vi "Read Commands.vi"(8 "error in (no error)":errorcluster, 11 "Iteration Actions in":refnum<class "Iteration Actions.lvclass">) -> (0 "error out":errorcluster, 1 "Analog Commands":map{refnum<class "MessageQ.lvclass">, T3}(c390), 2 "Digital Commands":map{refnum<class "MessageQ.lvclass">, T5}(c390), 3 "Iteration Actions out":refnum<class "Iteration Actions.lvclass">, 4 "Remote Analog":map{string, T1}(c390), 6 "Remote Digital":map{string, T2}(c390))   [LabVIEW 2020, in "VolatusSeq.lvlib" / "Iteration Actions.lvclass"]
uses:
  Iteration Actions.lvclass
  Volatus/MessageQ/MessageQ.lvclass
  messages/CmdDigitalMultiple/Data.ctl
  messages/CmdDigital/Data.ctl
  messages/CmdAnalogMultiple/Data.ctl
  messages/CmdAnalog/Data.ctl
  Iteration Actions.lvclass/Iteration Actions.ctl
  messages/CmdDigital/CmdDigital.lvlib
  messages/CmdDigitalMultiple/CmdDigitalMultiple.lvlib
  messages/CmdAnalog/CmdAnalog.lvlib
  messages/CmdAnalogMultiple/CmdAnalogMultiple.lvlib
  messages/CmdDigitalMultiple/Class/Msg.lvclass
  Remote Digital.ctl
  VolatusSeq.lvlib
  messages/CmdAnalogMultiple/Class/Msg.lvclass
  Remote Analog.ctl
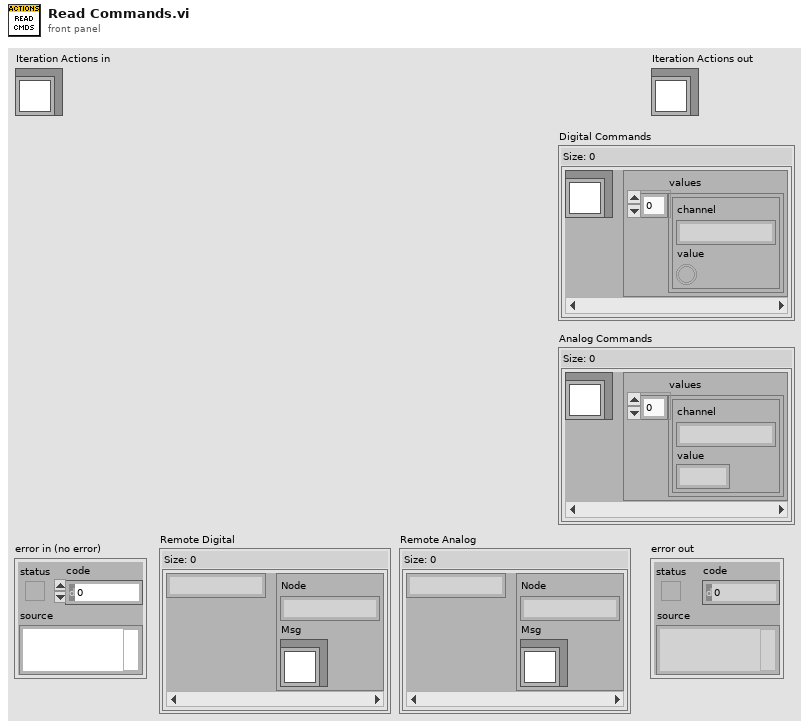
[diagram p1: front panel]
types:
  T1 = typedef "VolatusSeq.lvlib/Remote Analog.ctl" = cluster{"Node":string, "Msg":refnum<class "Msg.lvclass">}
  T2 = typedef "VolatusSeq.lvlib/Remote Digital.ctl" = cluster{"Node":string, "Msg":refnum<class "Msg.lvclass">}
  T3 = typedef "CmdAnalogMultiple.lvlib/Data.ctl" = cluster{"values":T4[]}
  T4 = typedef "CmdAnalog.lvlib/Data.ctl" = cluster{"channel":string, "value":dbl}
  T5 = typedef "CmdDigitalMultiple.lvlib/Data.ctl" = cluster{"values":T6[]}
  T6 = typedef "CmdDigital.lvlib/Data.ctl" = cluster{"channel":string, "value":bool}
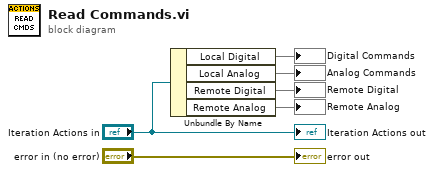
[diagram p0: block diagram]
diagram:
  n1 = Unbundle By Name("Iteration Actions in") -> ("Local Digital"=→"Digital Commands":map{refnum<class "MessageQ.lvclass">, T5}, "Local Analog"=→"Analog Commands":map{refnum<class "MessageQ.lvclass">, T3}, "Remote Digital"=→"Remote Digital":map{string, T2}, "Remote Analog"=→"Remote Analog":map{string, T1})
  "error out" <- "error in (no error)"
  "Iteration Actions out" <- "Iteration Actions in"
